vi "Get Stock Info.vi"(8 "error in":errorcluster) -> (0 "error out":errorcluster, 3 "Stocks":T1(array[cluster]))   [LabVIEW 2020, in "Full Featured MCP Server.lvlib"]
doc: "Returns every stock with its sector, a short company description, the current price in euros, the price change over the last 60 seconds in percent and how many shares you own. Read the descriptions: they tell you how solid a company is. Combine them with get_news and get_history_chart before you buy or sell."
uses:
  Full Featured MCP Server.lvlib
  Market/Market Mode.ctl
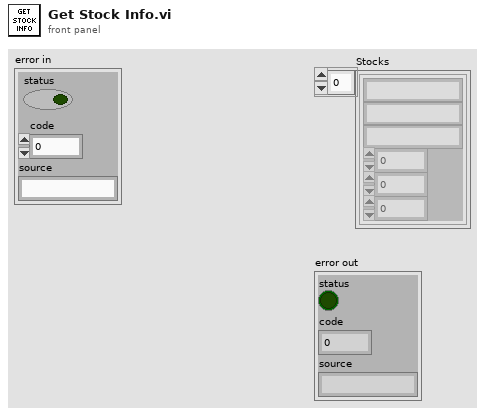
[diagram p1: front panel]
types:
  T1 = cluster{"name":string, "sector":string, "description":string, "price":dbl, "change_60s_percent":dbl, "owned":i32}[]
  T2 = typedef "Full Featured MCP Server.lvlib/Market Mode.ctl" = enum16{"Get", "Init", "Advance", "Buy", "Sell"}
  T3 = cluster{"name":string, "sector":i32, "quality":i32, "start price":dbl, "drift":dbl, "volatility":dbl, "beta":dbl, "jumpiness":dbl, "description":string}[]
  T4 = cluster{"tick":i32, "price history":dbl[][], "shock":dbl[], "momentum":dbl[], "nervousness":dbl[], "mood":dbl, "tension":dbl, "sector mood":dbl[], "news":cluster{"tick":i32, "headline":string, "stocks":i32[], "direction":string}[], "stories":cluster{"arc":i32, "step":i32, "due":i32, "stock":i32, "other":i32}[], "owned":i32[], "wallet":dbl}
  T5 = cluster{"name":string, "sector":string, "description":string, "price":dbl, "change_60s_percent":dbl, "owned":i32}
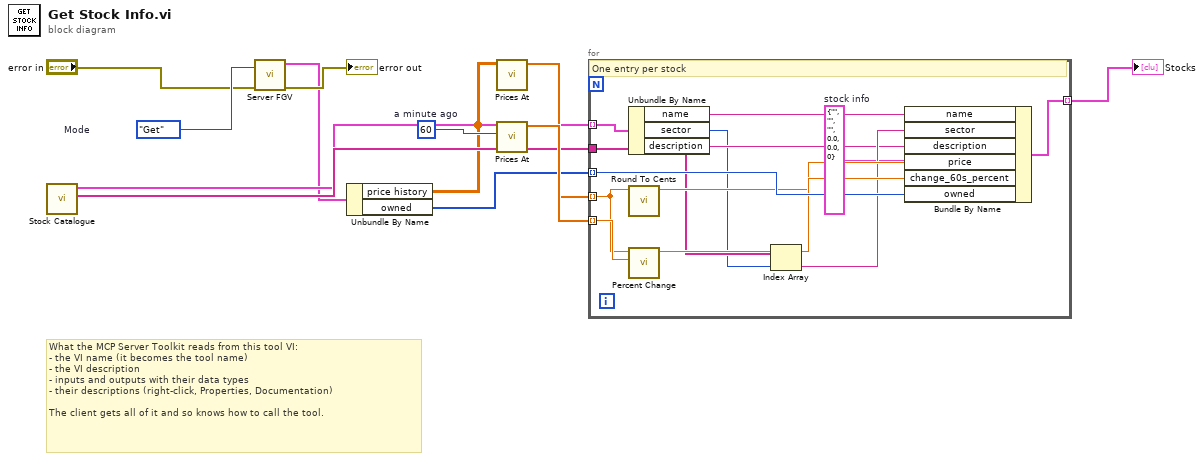
[diagram p0: block diagram]
diagram:
  w12 = 60  # a minute ago
  w2 = Market_Mode."Get"  # Mode
  # "What the MCP Server Toolkit reads from this tool VI:\n- the VI name (it becomes the tool name)\n- the VI description\n- inputs and outputs with their data types\n- their descriptions (right-click, Properties, Documentation)\n\nThe client gets all of it and so knows how to call the tool."
  n1 = call "Stock Catalogue.vi"() -> ("sectors"=w8:string[], "stocks"=w7:T3)  [unwired: 10 in]
  n2 = call "Server FGV.vi"("Mode"=w2, "error in"="error in") -> ("error out"=→"error out":errorcluster, "market"=w3:T4)  [unwired: 7 in, 1 out]
  n3 = Unbundle By Name(w3) -> ("price history"=w5:dbl[][], "owned"=w6:i32[])
  n4 = call "Prices At.vi"("price history"=w5) -> ("prices"=w9:dbl[])  [unwired: 10 in]
  n5 = call "Prices At.vi"("seconds ago"=w12, "price history"=w5) -> ("prices"=w10:dbl[])  [unwired: 9 in]
  n6 = for {
    tunnel: w7 -> [w13] mode=indexing
    tunnel: w8 -> [w20]
    tunnel: w6 -> [w24] mode=indexing
    tunnel: w9 -> [w17] mode=indexing
    tunnel: w10 -> [w18] mode=indexing
    tunnel: [w25] -> w11 mode=indexing
    w19 = T5 {"name"="", "sector"="", "description"="", "price"=0.0, "change_60s_percent"=0.0, "owned"=0}  # stock info
    # "One entry per stock"
    n7 = Unbundle By Name(w13) -> ("name"=w14:string, "sector"=w15:i32, "description"=w16:string)
    n8 = call "Round To Cents.vi"("amount"=w17) -> ("rounded"=w22:dbl)  [unwired: 10 in]
    n9 = call "Percent Change.vi"("before"=w18, "now"=w17) -> ("percent"=w23:dbl)  [unwired: 9 in]
    n10 = Index Array(array=w20, index=w15) -> (element=w21:string)
    n11 = Bundle By Name(cluster=w19, "name"=w14, "sector"=w21, "description"=w16, "price"=w22, "change_60s_percent"=w23, "owned"=w24) -> (w25:T5)
  }
  "Stocks" <- w11
